vi "PIDController_Execute.vi"(4 "PID Error Tolerance":T2={"PositionTolerance"=0.001, "VelocityTolerance"=9.9e+30}, 6 "Period":dbl=0.02, 7 "PID Input Limits":T1, 8 "Reset":bool, 9 "SP-SetPoint":dbl, 10 "PV-Measurement":dbl, 11 "PID Tuning":T3={"Kp"=0.0, "Ki"=0.0, "Kd"=0.0, "MaximumIntegral"=9.9e+30, "MinimumIntegral"=-9.9e+30, "IntegralZone"=9.9e+30}) -> (0 "AtSetpoint":bool, 1 "CO-ControlOutput":dbl, 3 "out PID_CONTROLLER":T4={"Kp"=0.0, "Ki"=0.0, "Kd"=0.0, "Period"=0.0, "Max_Integral"=0.0, "Min_Integral"=0.0, "Max_Input"=0.0, "Min_Input"=0.0, "Continuous"=FALSE, "PositionError"=0.0, "VelocityError"=0.0, "PrevError"=0.0, "Total_Integral"=0.0, "PositionTolerance"=0.0, "VelocityTolerance"=0.0, "SetPoint"=0.0, "Kf"=0.0, "Prev_Deriv"=0.0, "Prev_Deriv 2"=0.0, "DerivativeFilter"=FALSE, "Min_Output"=-9.99e+35, "Max_Output"=9.9e+35, "Prev_F_P"=0.0, "Prev_F_P_2"=0.0, "AntiWindupActive"=FALSE, "Measurement"=0.0, "IntegralZone"=9.9e+30} {"IntegralZone" format="%16_6e"; "Measurement" format="%16_6e"; "Prev_F_P_2" format="%16_6e"; "Prev_F_P" format="%16_6e"; "Max_Output" format="%16_6e"; "Min_Output" format="%16_6e"; "Prev_Deriv 2" format="%16_6e"; "Prev_Deriv" format="%16_6e"; "Kf" format="%16_6e"; "SetPoint" format="%16_6e"; "VelocityTolerance" format="%16_6e"; "PositionTolerance" format="%16_6e"; "Total_Integral" format="%16_6e"; "PrevError" format="%16_6e"; "VelocityError" format="%16_6e"; "PositionError" format="%16_6e"; "Min_Input" format="%16_6e"; "Max_Input" format="%16_6e"; "Min_Integral" format="%16_6e"; "Max_Integral" format="%16_6e"; "Period" format="%16_6e"; "Kd" format="%16_6e"; "Ki" format="%16_6e"; "Kp" format="%16_6e"})   [LabVIEW 2019, in "Trajectory_Library.lvlib"]
doc: "Convience, single call, LabVIEW function. Creates and calculates the PID controller. Call this routine periodically to calculate the newest output for the provided inputs. \n \nInputs:\n - PID Input Limits -- Cluster containing:\n - MaxInput -- (Default: 0)\n - MinInput -- (Default: 0)\n - Continous -- When True indicates that the input is continuous. (Default: False)\n - PID Tuning -- PID Tuning parameters containing:\n - Kp -- The proportional coefficient.\n - Ki -- The integral coefficient.\n - Kd -- The derivative coefficient.\n - Maximum Integral -- The maximum value of the integrator.\n - Minimum Integral -- The minimum value of the integrator.\n - PV-measurement The current measurement of the process variable. (PV)\n - SP-setpoint The new setpoint of the controller. (SP)\n - Reset -- When True, causes the PID to be reset. (Default: False)\n - Period -- Period of repeated calls in seconds. (Default: 0.020)\n - PID Error Tolerance -- Tolerances for determining \"At Setpoint\", contains:\n - Position Tolerance -- (Default: 0.001)\n - Velocity Tolerance -- (Default: 9.9E+30)\nOutputs:\n - PID_Controller -- Updated PID_Controller data cluster\n - CO-ControlOutput -- Controller output (CO) \n - AtSetpoint -- True when PV is within the specified tolerances of the SP."
uses:
  Trajectory_Library.lvlib
  TypeDef/PID_CONTROLLER.ctl
  TypeDef/PID_TUNING.ctl
  TypeDef/PID_ERROR_TOLERANCE.ctl
  TypeDef/PID_INPUT_LIMITS.ctl
  PIDController_SetSetpoint.vi
  PIDController_Calculate_PV.vi
  <vilib>/Rock Robotics/SystemInterfaces/NetworkCommunication/NetComm_UsageReport_report.vi
  ControllerUtil_GetModulusError.vi
  Globals/Util_LibraryGlobals.vi
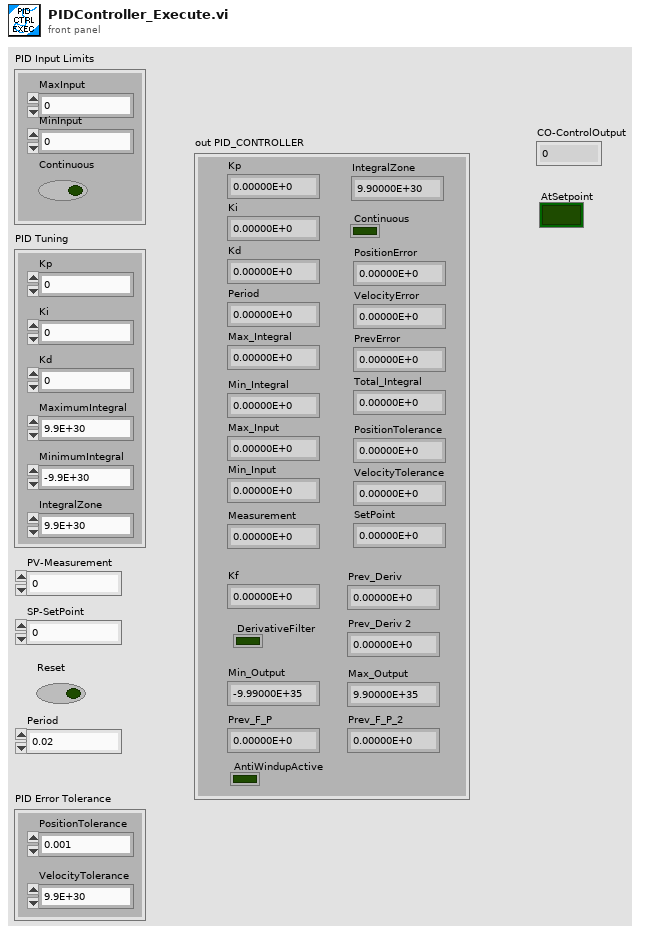
[diagram p1: front panel]
types:
  T1 = typedef "Trajectory_Library.lvlib/PID_INPUT_LIMITS.ctl" = cluster{"MaxInput":dbl, "MinInput":dbl, "Continuous":bool}
  T2 = typedef "Trajectory_Library.lvlib/PID_ERROR_TOLERANCE.ctl" = cluster{"PositionTolerance":dbl, "VelocityTolerance":dbl}
  T3 = typedef "Trajectory_Library.lvlib/PID_TUNING.ctl" = cluster{"Kp":dbl, "Ki":dbl, "Kd":dbl, "MaximumIntegral":dbl, "MinimumIntegral":dbl, "IntegralZone":dbl}
  T4 = typedef "Trajectory_Library.lvlib/PID_CONTROLLER.ctl" = cluster{"Kp":dbl, "Ki":dbl, "Kd":dbl, "Period":dbl, "Max_Integral":dbl, "Min_Integral":dbl, "Max_Input":dbl, "Min_Input":dbl, "Continuous":bool, "PositionError":dbl, "VelocityError":dbl, "PrevError":dbl, "Total_Integral":dbl, "PositionTolerance":dbl, "VelocityTolerance":dbl, "SetPoint":dbl, "Kf":dbl, "Prev_Deriv":dbl, "Prev_Deriv 2":dbl, "DerivativeFilter":bool, "Min_Output":dbl, "Max_Output":dbl, "Prev_F_P":dbl, "Prev_F_P_2":dbl, "AntiWindupActive":bool, "Measurement":dbl, "IntegralZone":dbl}
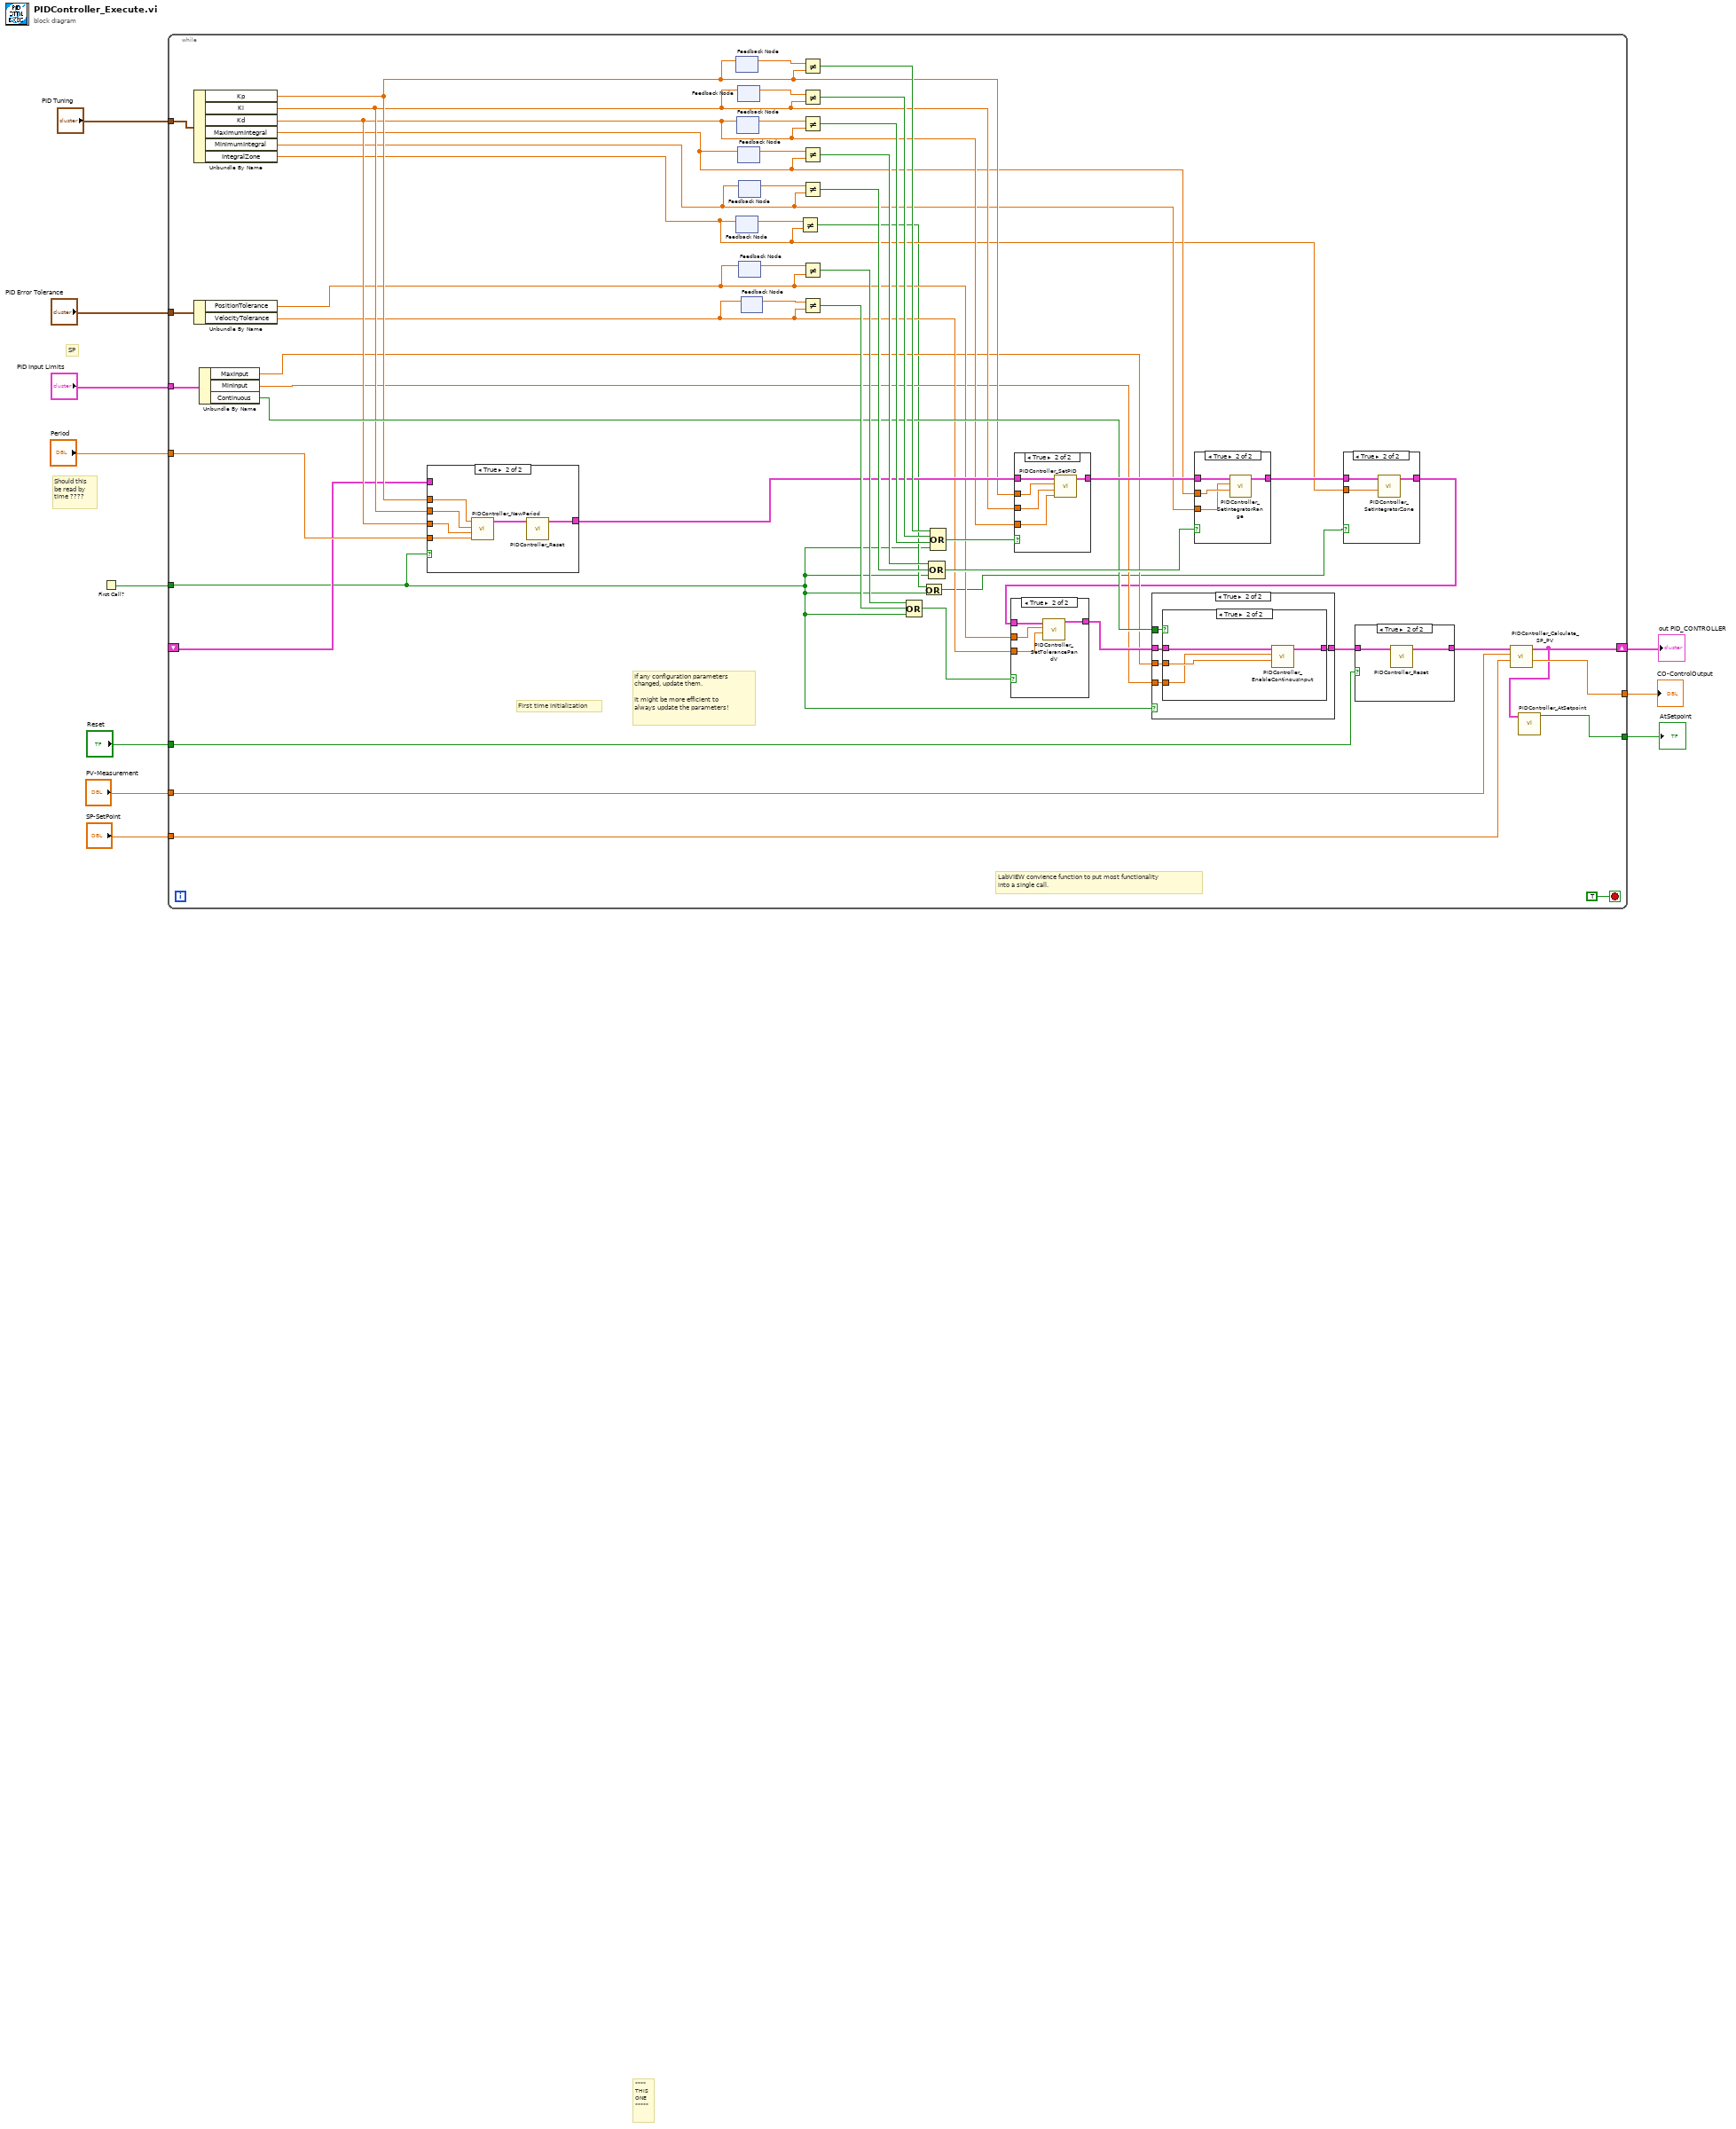
[diagram p0: block diagram]
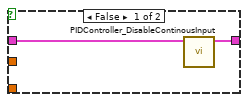
[diagram p6: hidden frame]
diagram:
  # "Should this\nbe read by\ntime ????"
  # "SP"
  # "****\nTHIS\nONE\n*****"
  n1 = First Call?() -> (First Call?: T/F=w4:bool)
  n2 = while {
    tunnel: [w62] -> w11
    tunnel: "PID Tuning" -> [w61]
    tunnel: [w60] -> w9
    tunnel: "PID Error Tolerance" -> [w59]
    tunnel: "PID Input Limits" -> [w58]
    tunnel: "Period" -> [w57]
    tunnel: w4 -> [w12]
    tunnel: "Reset" -> [w23]
    tunnel: "SP-SetPoint" -> [w22]
    tunnel: "PV-Measurement" -> [w21]
    shift-right: [w25] -> w5
    shift-left: _ -> [w20]
    stop <- TRUE stop-if-true
    # "First time initialization"
    # "If any configuration parameters \nchanged, update them.\n\nIt might be more efficient to\nalways update the parameters!"
    # "LabVIEW convience function to put most functionality\ninto a single call."
    n3 = Unbundle By Name(w61) -> ("Kp"=w41:dbl, "Ki"=w40:dbl, "Kd"=w39:dbl, "MaximumIntegral"=w38:dbl, "MinimumIntegral"=w37:dbl, "IntegralZone"=w16:dbl)
    n4 = Unbundle By Name(w59) -> ("PositionTolerance"=w36:dbl, "VelocityTolerance"=w35:dbl)
    n5 = Unbundle By Name(w58) -> ("MaxInput"=w34:dbl, "MinInput"=w33:dbl, "Continuous"=w42:bool)
    n6 = case shown="True" w12 {
      tunnel: w41 -> [_ w73]
      tunnel: w40 -> [_ w72]
      tunnel: w39 -> [_ w71]
      tunnel: w57 -> [_ w70]
      tunnel: [w67 w69] -> w43
      tunnel: w20 -> [w67 _]
      frame False {
      }
      frame True {
        n7 = call "PIDController_NewPeriod.vi"("Period"=w70, "Kd"=w71, "Ki"=w72, "Kp"=w73) -> ("PID_CONTROLLER"=w68:T4)  [unwired: 7 in]
        n8 = call "PIDController_Reset.vi"("in PID_CONTROLLER"=w68) -> ("out PID_CONTROLLER"=w69:T4)  [unwired: 10 in]
      }
    }
    n9 = feedback #1() -> (w32:dbl)  [unwired: 1 in]
    n10 = feedback-in #1(w41) -> ()
    n11 = feedback #2() -> (w19:dbl)  [unwired: 1 in]
    n12 = feedback-in #2(w16) -> ()
    n13 = feedback #3() -> (w30:dbl)  [unwired: 1 in]
    n14 = feedback-in #3(w39) -> ()
    n15 = feedback #4() -> (w31:dbl)  [unwired: 1 in]
    n16 = feedback-in #4(w40) -> ()
    n17 = feedback #5() -> (w29:dbl)  [unwired: 1 in]
    n18 = feedback-in #5(w38) -> ()
    n19 = feedback #6() -> (w28:dbl)  [unwired: 1 in]
    n20 = feedback-in #6(w37) -> ()
    n21 = feedback #7() -> (w27:dbl)  [unwired: 1 in]
    n22 = feedback-in #7(w36) -> ()
    n23 = feedback #8() -> (w26:dbl)  [unwired: 1 in]
    n24 = feedback-in #8(w35) -> ()
    n25 = Not Equal?(x=w19, y=w16) -> (x != y?=w13:bool)
    n26 = Not Equal?(x=w32, y=w41) -> (x != y?=w50:bool)
    n27 = Not Equal?(x=w31, y=w40) -> (x != y?=w51:bool)
    n28 = Not Equal?(x=w30, y=w39) -> (x != y?=w52:bool)
    n29 = Not Equal?(x=w29, y=w38) -> (x != y?=w53:bool)
    n30 = Not Equal?(x=w28, y=w37) -> (x != y?=w54:bool)
    n31 = Not Equal?(x=w27, y=w36) -> (x != y?=w55:bool)
    n32 = Not Equal?(x=w26, y=w35) -> (x != y?=w56:bool)
    n33 = Compound Arithmetic op=OR(w55, w56, w12) -> (w15:bool)
    n34 = Or(x=w13, y=w12) -> (x .or. y?=w14:bool)
    n35 = Compound Arithmetic op=OR(w53, w54, w12) -> (w47:bool)
    n36 = Compound Arithmetic op=OR(w50, w51, w52, w12) -> (w49:bool)
    n37 = case shown="True" w49 {
      tunnel: w43 -> [w99 w104]
      tunnel: w41 -> [_ w103]
      tunnel: w40 -> [_ w102]
      tunnel: w39 -> [_ w101]
      tunnel: [w99 w100] -> w48
      frame False {
      }
      frame True {
        n38 = call "PIDController_SetPID.vi"("Kd"=w101, "Ki"=w102, "Kp"=w103, "in PID_CONTROLLER"=w104) -> ("out PID_CONTROLLER"=w100:T4)  [unwired: 7 in]
      }
    }
    n39 = case shown="True" w47 {
      tunnel: w48 -> [w94 w98]
      tunnel: w38 -> [_ w97]
      tunnel: w37 -> [_ w96]
      tunnel: [w94 w95] -> w17
      frame False {
      }
      frame True {
        n40 = call "PIDController_SetIntegratorRange.vi"("MaximumIntegral"=w97, "MinimumIntegral"=w96, "in PID_CONTROLLER"=w98) -> ("out PID_CONTROLLER"=w95:T4)  [unwired: 8 in]
      }
    }
    n41 = case shown="True" w14 {
      tunnel: w17 -> [w63 w66]
      tunnel: [w63 w65] -> w18
      tunnel: w16 -> [_ w64]
      frame False {
      }
      frame True {
        n42 = call "PIDController_SetIntegratorZone.vi"("IntegratorZone"=w64, "in PID_CONTROLLER"=w66) -> ("out PID_CONTROLLER"=w65:T4)  [unwired: 9 in]
      }
    }
    n43 = case shown="True" w15 {
      tunnel: w18 -> [w89 w93]
      tunnel: w36 -> [_ w92]
      tunnel: w35 -> [_ w91]
      tunnel: [w89 w90] -> w46
      frame False {
      }
      frame True {
        n44 = call "PIDController_SetTolerancePandV.vi"("VelocityTolerance"=w91, "PositionTolerance"=w92, "in PID_CONTROLLER"=w93) -> ("out PID_CONTROLLER"=w90:T4)  [unwired: 8 in]
      }
    }
    n45 = case shown="True" w12 {
      tunnel: w34 -> [_ w82]
      tunnel: w33 -> [_ w81]
      tunnel: w46 -> [w77 w80]
      tunnel: w42 -> [_ w79]
      tunnel: [w77 w78] -> w45
      frame False {
      }
      frame True {
        n46 = case shown="True" w79 {
          tunnel: w80 -> [w84 w88]
          tunnel: [w83 w87] -> w78
          tunnel: w82 -> [_ w86]
          tunnel: w81 -> [_ w85]
          frame False {
            n47 = call "PIDController_DisableContinousInput.vi"("in PID_CONTROLLER"=w84) -> ("out PID_CONTROLLER"=w83:T4)  [unwired: 10 in]
          }
          frame True {
            n48 = call "PIDController_EnableContinousInput.vi"("MaxInput"=w86, "MinInput"=w85, "in PID_CONTROLLER"=w88) -> ("out PID_CONTROLLER"=w87:T4)  [unwired: 8 in]
          }
        }
      }
    }
    n49 = case shown="True" w23 {
      tunnel: w45 -> [w74 w76]
      tunnel: [w74 w75] -> w44
      frame False {
      }
      frame True {
        n50 = call "PIDController_Reset.vi"("in PID_CONTROLLER"=w76) -> ("out PID_CONTROLLER"=w75:T4)  [unwired: 10 in]
      }
    }
    n51 = call "PIDController_Calculate_SP_PV.vi"("SP-SetPoint"=w22, "PV-Measurement"=w21, "in PID_CONTROLLER"=w44) -> ("CO-ControlOutput"=w62:dbl, "out PID_CONTROLLER"=w25:T4)  [unwired: 7 in]
    n52 = call "PIDController_AtSetpoint.vi"("in PID_CONTROLLER"=w25) -> ("AtSetpoint"=w60:bool)  [unwired: 10 in]
  }
  "out PID_CONTROLLER" <- w5
  "CO-ControlOutput" <- w11
  "AtSetpoint" <- w9
